vi "Write.vi"(6 "write to Cache only? (F)":bool, 7 "Qualified Name":string, 8 "error in (no error)":errorcluster, 9 "Values":variant[](array[variant]), 10 "keys":string[](array[string]), 11 "ConfigManager in":refnum<class "ConfigManager.lvclass">) -> (0 "error out":errorcluster, 2 "keys dup":string[](array[string]), 3 "ConfigManager out":refnum<class "ConfigManager.lvclass">)   [LabVIEW 2013, in "CfgManager.lvlib" / "ConfigManager.lvclass"]
uses:
  ConfigManager.lvclass
  <vilib>/Utility/VariantDataType/VariantType.lvlib
  Encoding/Encoding.lvclass
  Serializer/Serializer.lvclass
  Encryption/Encryption.lvclass
  Cache/ConfigManager.Cache.lvclass
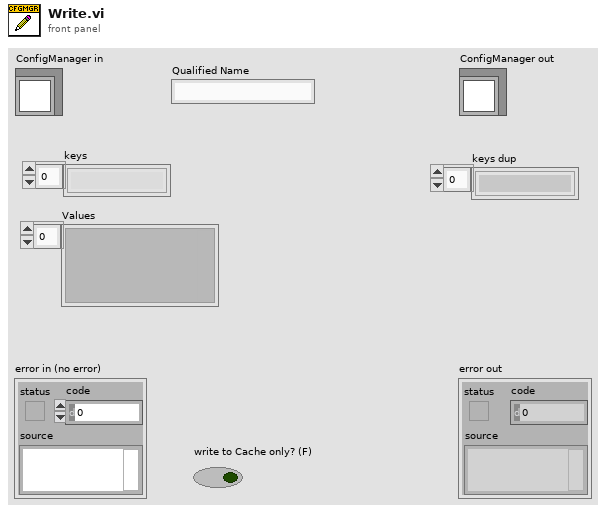
[diagram p1: front panel]
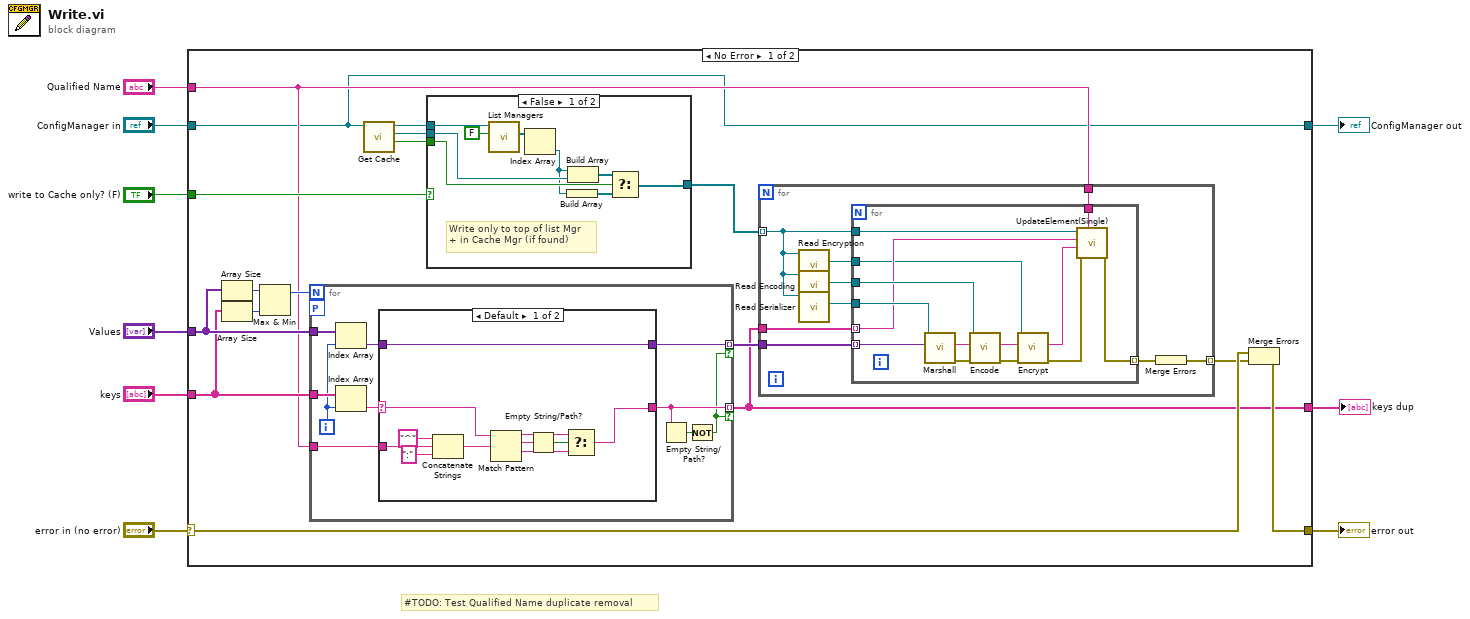
[diagram p0: block diagram]
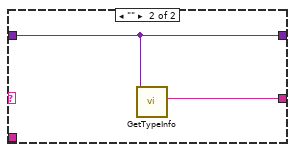
[diagram p2: hidden frame]
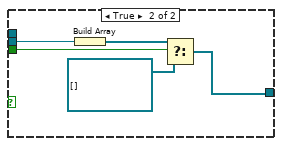
[diagram p3: hidden frame]
diagram:
  # "#TODO: Test Qualified Name duplicate removal"
  n1 = case shown="No Error" "error in (no error)" {
    selector: "error in (no error)" -> [w26 w87]
    tunnel: [w25 w87] -> w6
    tunnel: [w10 w86] -> w8
    tunnel: "ConfigManager in" -> [w10 w86]
    tunnel: "keys" -> [w14 w85]
    tunnel: "Values" -> [w15 _]
    tunnel: [w12 w85] -> w3
    tunnel: "Qualified Name" -> [w11 _]
    tunnel: "write to Cache only? (F)" -> [w19 _]
    frame No Error {
      n2 = Array Size(array=w15) -> (size(s)=w21:i32)
      n3 = Array Size(array=w14) -> (size(s)=w23:i32)
      n4 = Max & Min(x=w21, y=w23) -> (max(x,y)=w16:i32)  [unwired: 1 out]
      n5 = for {
        N: w16 -> [_]
        tunnel: w15 -> [w34]
        tunnel: w14 -> [w33]
        tunnel: [w31] -> w13 mode=indexing if=w28
        tunnel: [w30] -> w12 mode=indexing if=w28
        tunnel: w11 -> [w27]
        workers-P: _ -> [_]
        i -> [w32]
        n6 = Index Array(array=w34, index=w32) -> (element=w35:variant)
        n7 = Index Array(array=w33, index=w32) -> (element=w36:string)
        n8 = case shown="Default" w36 {
          selector: w36 -> [w38 _]
          tunnel: w35 -> [w47 w48]
          tunnel: [w37 w49] -> w30
          tunnel: [w47 w48] -> w31
          tunnel: w27 -> [w39 _]
          frame Default {
            n9 = Concatenate Strings("^" ("string"), w39, ":" ("string")) -> (w40:string)
            n10 = Match Pattern(string=w38, regular expression=w40) -> (before substring=w44:string, match substring=w42:string, after substring=w45:string)  [unwired: 1 in, 1 out]
            n11 = Empty String/Path?(string/path=w42) -> (empty?=w43:bool)
            n12 = Select(t=w44, s=w43, f=w45) -> (s? t:f=w37:string)
          }
          frame "" {
            n13 = call <vilib>:"GetTypeInfo.vi"("Variant"=w48) -> ("Name"=w49:string)  [unwired: 6 in, 4 out]
          }
        }
        n14 = Empty String/Path?(string/path=w30) -> (empty?=w29:bool)
        n15 = Not(x=w29) -> (.not. x?=w28:bool)
      }
      n16 = call-dynamic "Get Cache.vi"("ConfigManager in"=w10) -> ("found?"=w20:bool, "Cache"=w18:refnum<class "ConfigManager.Cache.lvclass">, "ConfigManager out"=w22:refnum<class "ConfigManager.lvclass">)  [unwired: 8 in]
      n17 = case shown="False" w19 {
        tunnel: [w74 w81] -> w17
        tunnel: w22 -> [w78 _]
        tunnel: w20 -> [w75 w83]
        tunnel: w18 -> [w76 w84]
        frame False {
          # "Write only to top of list Mgr\n+ in Cache Mgr (if found)"
          n18 = call-dynamic "List Managers.vi"("Include Cache? (F)"=FALSE, "ConfigManager in"=w78) -> ("List"=w71:refnum<class "ConfigManager.lvclass">[])  [unwired: 8 in, 1 out]
          n19 = Index Array(array=w71) -> (element=w72:refnum<class "ConfigManager.lvclass">)  [unwired: 1 in]
          n20 = Build Array(w72) -> (w73:refnum<class "ConfigManager.lvclass">[])
          n21 = Build Array(w72, w76) -> (w77:refnum<class "ConfigManager.lvclass">[])
          n22 = Select(t=w77, s=w75, f=w73) -> (s? t:f=w74:refnum<class "ConfigManager.lvclass">[])
        }
        frame True {
          n23 = Build Array(w84) -> (w82:refnum<class "ConfigManager.Cache.lvclass">[])
          n24 = Select(t=w82, s=w83, f=refnum<class "ConfigManager.Cache.lvclass">[] []) -> (s? t:f=w81:refnum<class "ConfigManager.Cache.lvclass">[])
        }
      }
      n25 = for {
        tunnel: [w50] -> w24 mode=indexing
        tunnel: w11 -> [w55]
        tunnel: w13 -> [w54]
        tunnel: w12 -> [w53]
        tunnel: w17 -> [w51] mode=indexing
        n26 = call "Read Encryption.vi"("ConfigManager in"=w51) -> ("Encryption"=w52:refnum<class "Encryption.lvclass">)  [unwired: 9 in, 1 out]
        n27 = call "Read Encoding.vi"("ConfigManager in"=w51) -> ("Encoding"=w58:refnum<class "Encoding.lvclass">)  [unwired: 9 in, 1 out]
        n28 = call "Read Serializer.vi"("ConfigManager in"=w51) -> ("Serializer"=w57:refnum<class "Serializer.lvclass">)  [unwired: 9 in, 1 out]
        n29 = for {
          tunnel: w57 -> [w65]
          tunnel: w58 -> [w69]
          tunnel: [w66] -> w56 mode=indexing
          tunnel: w54 -> [w63] mode=indexing
          tunnel: w51 -> [w68]
          tunnel: w53 -> [w62] mode=indexing
          tunnel: w55 -> [w64]
          tunnel: w52 -> [w59]
          n30 = call-dynamic "Marshall.vi"("Variant"=w63, "Serializer in"=w65) -> ("error out"=w67:errorcluster, "String"=w70:string)  [unwired: 7 in, 1 out]
          n31 = call-dynamic "Encode.vi"("String"=w70, "CfgEncoding in"=w69) -> ("Encoded String"=w61:string)  [unwired: 8 in, 1 out]
          n32 = call-dynamic "Encrypt.vi"("String"=w61, "Encryption in"=w59) -> ("Encrypted String"=w60:string)  [unwired: 8 in, 1 out]
          n33 = call-dynamic "UpdateElement(Single).vi"("Qualified Name"=w64, "error in (no error)"=w67, "Value"=w60, "Key"=w62, "ConfigManager in"=w68) -> ("error out"=w66:errorcluster)  [unwired: 5 in, 1 out]
        }
        n34 = Merge Errors(w56) -> (w50:errorcluster)
      }
      n35 = Merge Errors(w26, w24) -> (w25:errorcluster)
    }
    frame Error {
    }
  }
  "error out" <- w6
  "ConfigManager out" <- w8
  "keys dup" <- w3
